vi "VIH - CHM Project - HHP Support - Get Key List.vi"(7 "Section":string, 8 "error in":errorcluster, 11 "queue":T1) -> (0 "error out":errorcluster, 2 "Keys":string[](array[string]), 3 "dup queue":T1)   [LabVIEW 2014]
doc: "::: VI Helpeks :::\nCopyright (c) 2000-2026 Konstantin Shifershteyn. All rights reserved."
uses:
  VIH - CHM Project - HHP Support - Queue Refnum.ctl
  VIH - CHM Project - HHP Support - Config Data Cluster.ctl
panel:
  # "VI Helpeks\nCopyright (c) 2012-2026 Konstantin Shifershteyn"
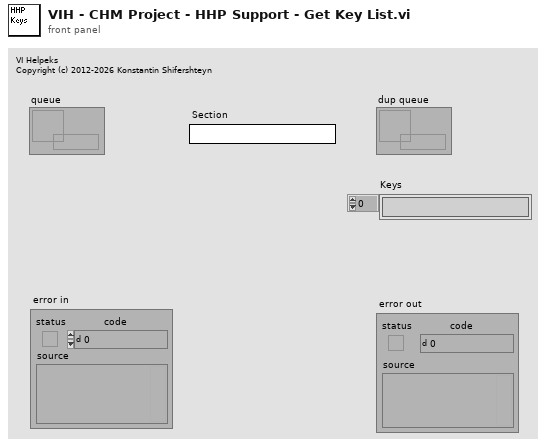
[diagram p1: front panel]
types:
  T1 = typedef "VIH - CHM Project - HHP Support - Queue Refnum.ctl" = refnum<queue>
  T2 = typedef "VIH - CHM Project - HHP Support - Config Data Cluster.ctl" = cluster{"Fille path":path, "sections":cluster{"Sec name":string, "key-values":string[][]}[]}
  T3 = cluster{"Sec name":string, "key-values":string[][]}[]
  T4 = cluster{"Sec name":string, "key-values":string[][]}
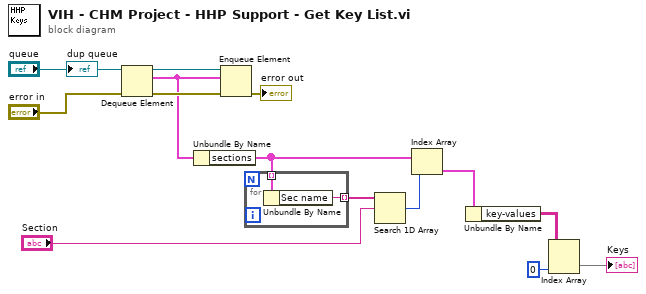
[diagram p0: block diagram]
diagram:
  n1 = Dequeue Element(queue="queue", error in (no error)="error in") -> (queue out=w14:T1, element=w2:T2, error out=w11:errorcluster)  [unwired: 1 in, 1 out]
  n2 = Unbundle By Name(w2) -> ("sections"=w6:T3)
  n3 = Enqueue Element(queue=w14, element=w2, error in (no error)=w11) -> (error out=→"error out":errorcluster)  [unwired: 1 in, 2 out]
  n4 = for {
    tunnel: w6 -> [w16] mode=indexing
    tunnel: [w15] -> w8 mode=indexing
    n5 = Unbundle By Name(w16) -> ("Sec name"=w15:string)
  }
  n6 = Search 1D Array(1D array=w8, element="Section") -> (index of element=w7:i32)  [unwired: 1 in]
  n7 = Index Array(array=w6, index=w7) -> (element=w4:T4)
  n8 = Unbundle By Name(w4) -> ("key-values"=w3:string[][])
  n9 = Index Array(array=w3, index (col)=0 ("disabled index (col)")) -> (element=→"Keys":string[])  [unwired: 1 in]
  "dup queue" <- "queue"
